vi "Create-Destroy.vi"(7 "Address":string, 8 "Error In":errorcluster) -> (0 "Error Out":errorcluster)   [LabVIEW 2018, in "Tests.lvlib" / "Known Hosts.lvlib"]
uses:
  Known Hosts.lvlib
  src/Toolkit/Known Hosts/Support/Create from Session.vi
  src/Toolkit/Known Hosts/Support/Destroy to Session.vi
  <vilib>/addons/_JKI Toolkits/Caraya/classes/Test/Test.lvclass
  <vilib>/addons/_JKI Toolkits/Caraya/classes/Assert/Assert.lvclass
  src/Toolkit/Known Hosts/Known Hosts.lvclass
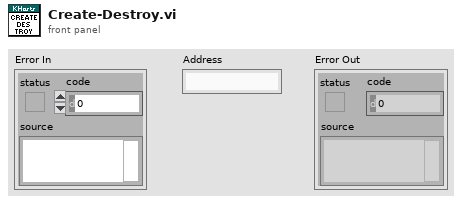
[diagram p1: front panel]
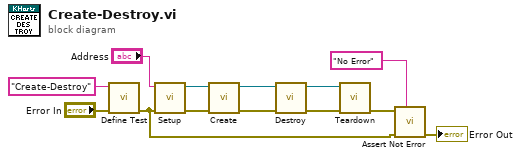
[diagram p0: block diagram]
diagram:
  n1 = call <vilib>:"Define Test.vi"("error in (no error)"="Error In", "Label (VI Title)"="Create-Destroy") -> ("error out"=w8:errorcluster)  [unwired: 9 in]
  n2 = call "Setup.vi"("Error In"=w8, "Address In"="Address") -> ("Error Out"=w5:errorcluster, "Sesssion"=w6:refnum<class "Session.lvclass">)  [unwired: 7 in, 1 out]
  n3 = call-poly "Create.vi"("Error In"=w5, "Session"=w6) -> ("Error Out"=w3:errorcluster, "Known Hosts"=w4:refnum<class "Known Hosts.lvclass">)  [unwired: 8 in]
  n4 = call-poly "Destroy.vi"("Error In"=w3, "Known Hosts"=w4) -> ("Error Out"=w1:errorcluster, "Session"=w2:refnum<class "Session.lvclass">)  [unwired: 8 in]
  n5 = call "Teardown.vi"("Error In"=w1, "Session"=w2) -> ("Error Out"=w11:errorcluster)  [unwired: 9 in]
  n6 = call <vilib>:"Assert Not Error.vi"("Label"="No Error", "error in (no error)"=w8, "Not Error?"=w11) -> ("error out"=→"Error Out":errorcluster)  [unwired: 8 in]
